vi "Match Key Regex.vi"(8 "error in":errorcluster, 10 "Datatype":T1, 11 "key in":string) -> (0 "error out":errorcluster, 1 "Datatype Found?":bool, 2 "Label out":string, 3 "key out":string)   [LabVIEW 2019, in "Instrument.Lockin.lvlib" / "Instrument.Lockin.lvclass"]
uses:
  Instrument.Lockin.lvclass
  Typedefs/Results Type--Enum.ctl
  <vilib>/regexp/Match Regular Expression.xnode
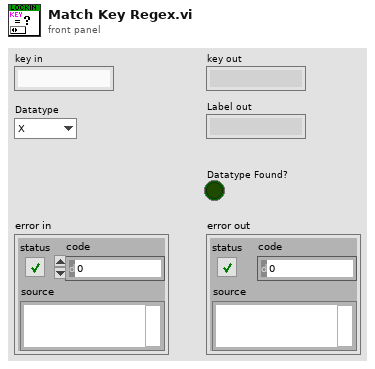
[diagram p1: front panel]
types:
  T1 = typedef "Instrument.Lockin.lvlib/Instrument.Lockin.lvclass/Results Type--Enum.ctl" = enum16{"X", "Y", "R", "Theta", "Mean"}
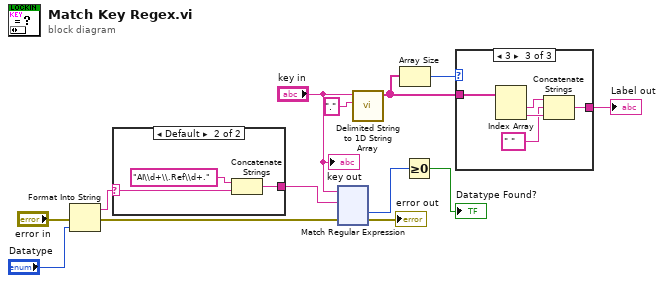
[diagram p0: block diagram]
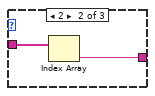
[diagram p3: hidden frame]
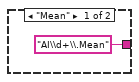
[diagram p4: hidden frame]
diagram:
  n1 = Format Into String(error in="error in", "Datatype") -> (resulting string=w10:string, error out=w6:errorcluster)  [unwired: 2 in]
  n2 = case shown="Default" w10 {
    selector: w10 -> [_ w16]
    tunnel: ["AI\\d+\\.Mean" ("regular expression") w15] -> w13
    frame "Mean" {
    }
    frame Default {
      n3 = Concatenate Strings("AI\\d+\\.Ref\\d+." ("regular expression"), w16) -> (w15:string)
    }
  }
  n4 = xnode "Match Regular Expression"("input string"="key in", "regular expression"=w13, "error in"=w6) -> ("offset past match"=w12:i32, "error out"=→"error out":errorcluster)  [unwired: 3 in, 3 out]
  n5 = call <vilib>:"Delimited String to 1D String Array.vi"("delimiter"=".", "delimited string"="key in") -> ("string array"=w3:string[])  [unwired: 9 in]
  n6 = Array Size(array=w3) -> (size(s)=w4:i32)
  n7 = Greater Or Equal To 0?(x=w12) -> (x >= 0?=→"Datatype Found?":bool)
  n8 = case shown="3" w4 {
    tunnel: w3 -> [_ w19 w24]
    tunnel: [_ w18 w23] -> w1
    frame Default {
    }
    frame 2 {
      n9 = Index Array(array=w19) -> (element=w18:string)  [unwired: 1 in]
    }
    frame 3 {
      n10 = Index Array(array=w24) -> (element #1=w22:string, element #2=w21:string)  [unwired: 2 in]
      n11 = Concatenate Strings(w22, " " ("string"), w21) -> (w23:string)
    }
  }
  "Label out" <- w1
  "key out" <- "key in"
